vi "CE Server - Build TCPAcessList.vi"(1 "TCPAccessList in":string[](array[string])) -> (0 "TCPAccessList out":string[](array[string]))   [LabVIEW 2021]
doc: "::: CalcExpress Toolkit :::\nCopyright (c) 2000-2026 Konstantin Shifershteyn. All rights reserved."
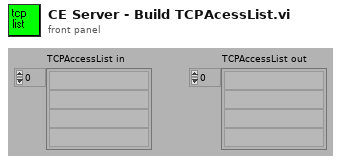
[diagram p1: front panel]
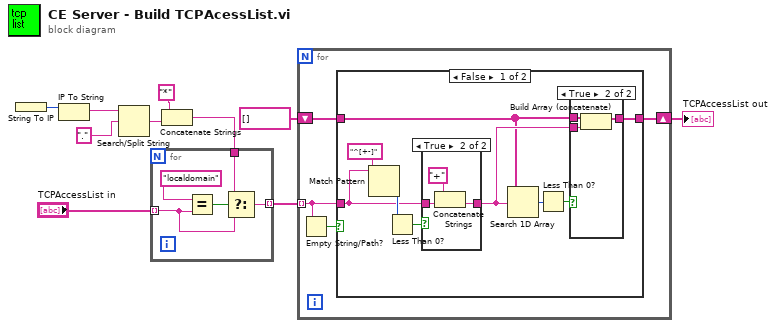
[diagram p0: block diagram]
diagram:
  n1 = String To IP() -> (0:w5:u32)  [unwired: 1 in]
  n2 = IP To String(2:w5) -> (0:w6:string)  [unwired: 1 in]
  n3 = Search/Split String(string=w6, search string/char (-)="." ("search char (-)")) -> (match + rest of string=w9:string)  [unwired: 1 in, 2 out]
  n4 = Concatenate Strings("*" ("search char (-)"), w9) -> (w10:string)
  n5 = for {
    tunnel: "TCPAccessList in" -> [w12] mode=indexing
    tunnel: w10 -> [w13]
    tunnel: [w11] -> w3 mode=indexing
    n6 = Equal?(x="localdomain", y=w12) -> (x = y?=w14:bool)
    n7 = Select(t=w13, s=w14, f=w12) -> (s? t:f=w11:string)
  }
  n8 = for {
    shift-right: [w17] -> w1
    shift-left: string[] [] -> [w19]
    tunnel: w3 -> [w18] mode=indexing
    n9 = Empty String/Path?(string/path=w18) -> (empty?=w16:bool)
    n10 = case shown="False" w16 {
      tunnel: w19 -> [w21 w37]
      tunnel: w18 -> [w24 _]
      tunnel: [w28 w37] -> w17
      frame False {
        n11 = Match Pattern(string=w24, regular expression="^[+-]") -> (offset past match=w26:i32)  [unwired: 1 in, 3 out]
        n12 = Less Than 0?(x=w26) -> (x < 0?=w25:bool)
        n13 = case shown="True" w25 {
          tunnel: [w33 w35] -> w22
          tunnel: w24 -> [w33 w36]
          frame False {
          }
          frame True {
            n14 = Concatenate Strings("+", w36) -> (w35:string)
          }
        }
        n15 = Search 1D Array(1D array=w21, element=w22) -> (index of element=w23:i32)  [unwired: 1 in]
        n16 = Less Than 0?(x=w23) -> (x < 0?=w20:bool)
        n17 = case shown="True" w20 {
          tunnel: [w29 w32] -> w28
          tunnel: w22 -> [_ w31]
          tunnel: w21 -> [w29 w30]
          frame False {
          }
          frame True {
            n18 = Build Array (concatenate)(w30, w31) -> (w32:string[])
          }
        }
      }
      frame True {
      }
    }
  }
  "TCPAccessList out" <- w1
